vi "Func - Unflatten-From-String Error handler.vi"(5 "InstanceRef":T1, 6 "error in":bool, 8 "argument number":i32=-1, 9 "Unflatten Error status":bool) -> (0 "error out":bool)   [LabVIEW 2021]
doc: "This VI handles an error produced by the <b>Unflatten From String</b> LabVIEW function. Refer to the VI help for more details.\n\n<b>argument number</b> control specifies the argument number where an unflattening error occurs. The VI adds the argument number to the error description to simplify debugging.\n\n<b>Unflatten Error status</b> control must be TRUE if an unflattening error occurred.\n\n::: CalcExpress Toolkit :::\nCopyright (c) 2000-2026 Konstantin Shifershteyn. All rights reserved."
uses:
  cetypes.llb/CalcExpress Instance RefNum.ctl
panel:
  out "error cluster out":errorcluster
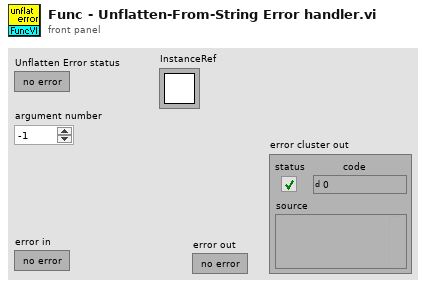
[diagram p1: front panel]
types:
  T1 = typedef "CalcExpress Instance RefNum.ctl" = refnum<k1>
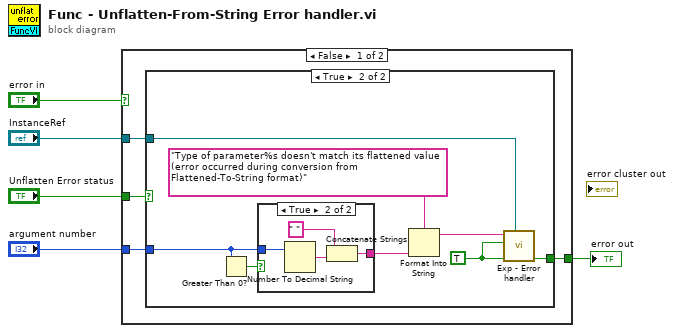
[diagram p0: block diagram]
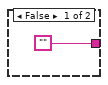
[diagram p3: hidden frame]
diagram:
  n1 = case shown="False" "error in" {
    selector: "error in" -> [_ w24]
    tunnel: [w9 w24] -> w5
    tunnel: "Unflatten Error status" -> [w8 _]
    tunnel: "InstanceRef" -> [w7 _]
    tunnel: "argument number" -> [w6 _]
    frame False {
      n2 = case shown="True" w8 {
        selector: w8 -> [w10 _]
        tunnel: [w10 w13] -> w9
        tunnel: w7 -> [_ w12]
        tunnel: w6 -> [_ w11]
        frame False {
        }
        frame True {
          w14 = TRUE ("error in")
          n3 = Greater Than 0?(x=w11) -> (x > 0?=w17:bool)
          n4 = case shown="True" w17 {
            tunnel: w11 -> [_ w21]
            tunnel: ["" w20] -> w16
            frame False {
            }
            frame True {
              n5 = Number To Decimal String(number=w21) -> (decimal integer string=w22:string)  [unwired: 1 in]
              n6 = Concatenate Strings(" ", w22) -> (w20:string)
            }
          }
          n7 = Format Into String(format string="Type of parameter%s doesn't match its flattened value (error occurred during conversion from Flattened-To-String format)", w16) -> (resulting string=w15:string)  [unwired: 2 in, 1 out]
          n8 = call "Exp - Error handler.vi"("InstanceRef"=w12, "error in"=w14, "add FuncName (T)"=w14, "error message in"=w15) -> ("error out"=w13:bool)  [unwired: 5 in, 2 out]
        }
      }
    }
    frame True {
    }
  }
  "error out" <- w5
